vi "Laser Power Ctrl Set Caption.vi"(2 "Caption Text":string, 7 "Setup Controls":refnum<vi>[](array[refnum])) -> ()   [LabVIEW 2016]
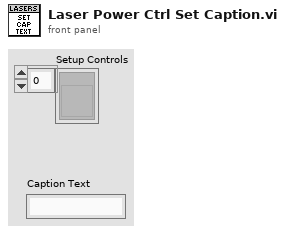
[diagram p1: front panel]
types:
  T1 = enum8{"Enabled", "Disabled", "Disabled and Grayed Out"}
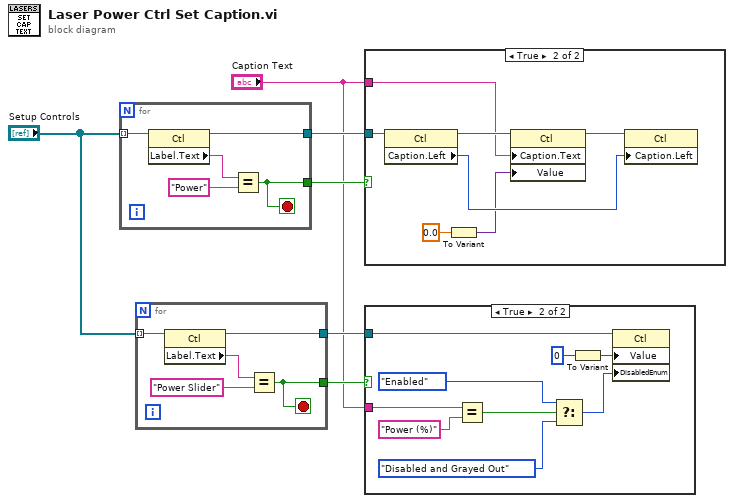
[diagram p0: block diagram]
diagram:
  n1 = for {
    tunnel: "Setup Controls" -> [w11] mode=indexing
    tunnel: [w8] -> w6
    tunnel: [w7] -> w5
    stop <- w8 stop-if-true
    n2 = property class="Ctl"(reference=w11) -> (reference out=w7:refnum<vi>, "Label.Text"=w10:string)  [unwired: 1 in, 1 out]
    n3 = Equal?(x=w10, y="Power") -> (x = y?=w8:bool)
  }
  n4 = for {
    tunnel: "Setup Controls" -> [w16] mode=indexing
    tunnel: [w13] -> w3
    tunnel: [w12] -> w2
    stop <- w13 stop-if-true
    n5 = property class="Ctl"(reference=w16) -> (reference out=w12:refnum<vi>, "Label.Text"=w15:string)  [unwired: 1 in, 1 out]
    n6 = Equal?(x=w15, y="Power Slider") -> (x = y?=w13:bool)
  }
  n7 = case shown="True" w6 {
    tunnel: w5 -> [_ w23]
    tunnel: "Caption Text" -> [_ w17]
    frame False {
    }
    frame True {
      n8 = property class="Ctl"(reference=w23) -> (reference out=w22:refnum<vi>, "Caption.Left"=w20:i32)  [unwired: 1 in, 1 out]
      n9 = To Variant(anything=0.0) -> (Variant=w19:variant)
      n10 = property class="Ctl"(reference=w22, "Caption.Text"=w17, "Value"=w19) -> (reference out=w21:refnum<vi>)  [unwired: 1 in, 1 out]
      n11 = property class="Ctl"(reference=w21, "Caption.Left"=w20) -> ()  [unwired: 1 in, 2 out]
    }
  }
  n12 = case shown="True" w3 {
    tunnel: w2 -> [_ w32]
    tunnel: "Caption Text" -> [_ w29]
    frame False {
    }
    frame True {
      n13 = Equal?(x=w29, y="Power (%)") -> (x = y?=w27:bool)
      n14 = Select(t=T1."Enabled" ("Disabled"), s=w27, f=T1."Disabled and Grayed Out") -> (s? t:f=w24:T1)
      n15 = To Variant(anything=u8 0) -> (Variant=w30:variant)
      n16 = property class="Ctl"(reference=w32, "Value"=w30, "DisabledEnum"=w24) -> ()  [unwired: 1 in, 2 out]
    }
  }
